vi "Prompt for Step.vi"(1 "Steps":T3[](array[typedef]), 3 "Index":i32=-1, 5 "error in (no error)":errorcluster) -> (16 "New Data Out":T3={"Type"=enum."Mouse Move", "X"=0, "Y"=0, "Delay"=0, "Key"=65, "Repeat"=0, "RClick?"=FALSE, "App/Window Name"="", "Notes"=""}, 18 "OK?":bool caption="OK", 19 "error out":errorcluster)   [LabVIEW 2023]
doc: "Prompts to enter a new step in the profile."
uses:
  CTLs/Step V3.ctl
  CTLs/Step Type V3.ctl
  <vilib>/Utility/inputDevices.llb/mouseAcquire.vi
  <vilib>/Utility/inputDevices.llb/closeMouse.vi
  <vilib>/Utility/config.llb/NI_LVConfig.lvlib
panel:
  in  "Save Default":bool
  in  "Step Notes":string
  out "Step Type Description":string
  in  "Repeat Amount":i32 min=0
  in  "Tab Control":T1(tab)
  in  "Y":i32 min=0
  in  "X":i32 min=0
  in  "Right Click?":bool
  in  "Key":u8(ring)=65
  in  "App/Window Name":string
  in  "Delay (ms)":i32=100 min=0
  in  "Step Type":T2
  in  "Cancel":bool
  in  "OK":bool caption="OK2"
  # "Left and right click at\nsame time to capture\ncurrent screen coords"
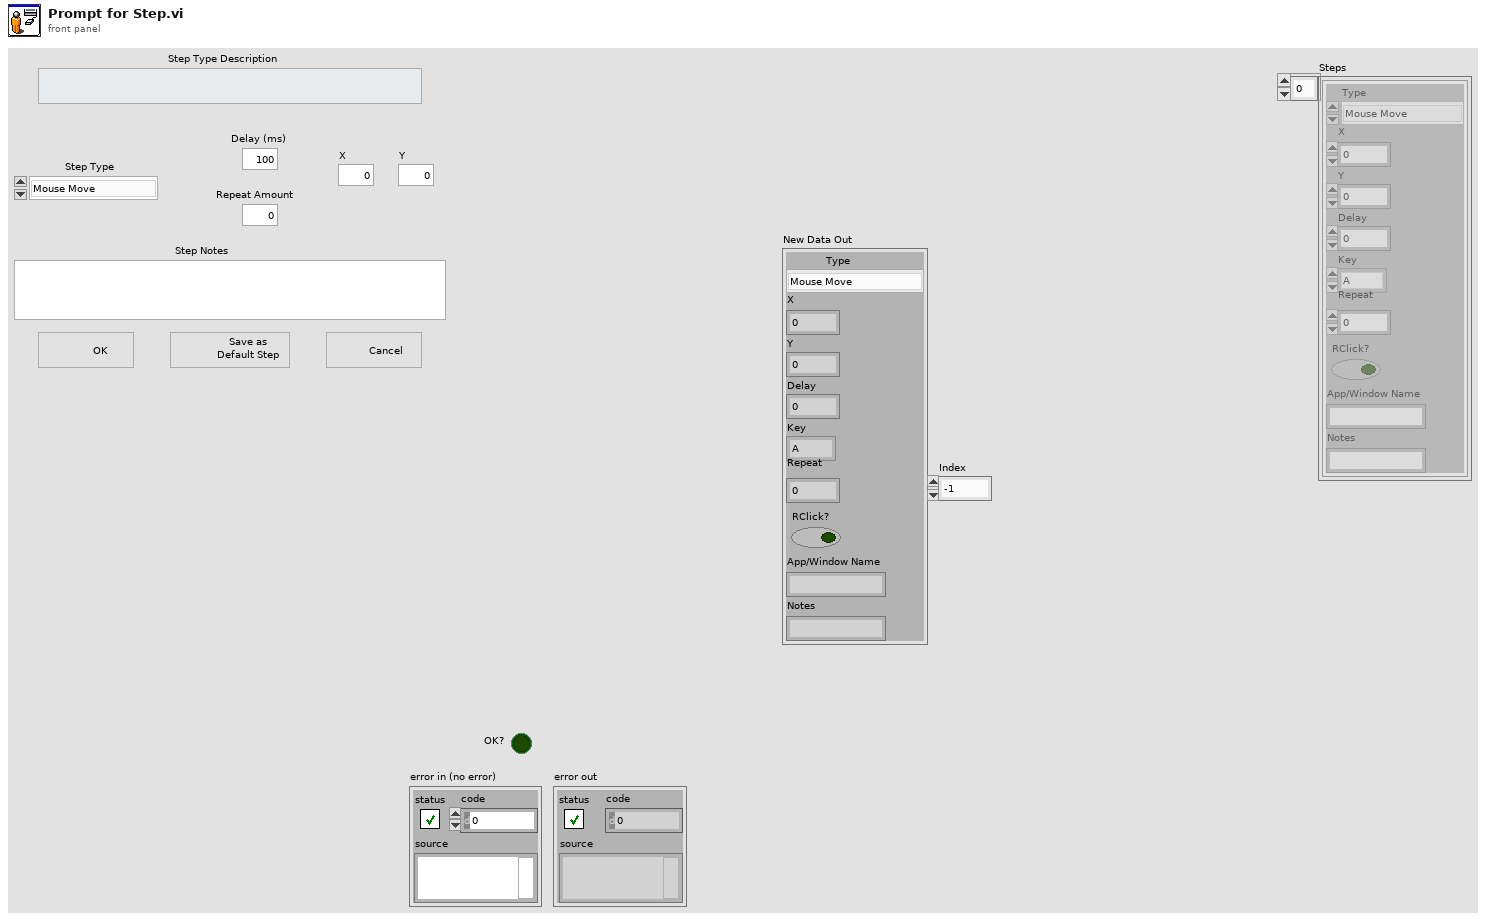
[diagram p1: front panel]
types:
  T1 = enum32{"Coords", "RClick", "Key", "A/W", "Nothing"}
  T2 = typedef "Step Type V3.ctl" = enum16{"Mouse Move", "Mouse Click", "Key Press", "Wait", "Mouse Down", "Mouse Up", "Key Down", "Key Up", "Run Application", "Maximize Window", "Restore Window", "Minimize Window", "Close Window", "Bring Window to Front", "Send Window to Back"}
  T3 = typedef "Step V3.ctl" = cluster{"Type":T2, "X":i32, "Y":i32, "Delay":i32, "Key":u8, "Repeat":i32, "RClick?":bool, "App/Window Name":string, "Notes":string}
  T4 = typedef "NI_LVConfig.lvlib/Config Data RefNum.ctl" = refnum<k1>
  T5 = cluster{"Horizontal":i32, "Vertical":i32, "Scrolling":i32}
  T6 = cluster{"button 1":bool, "button 2":bool, "button 3":bool, "button 4":bool}
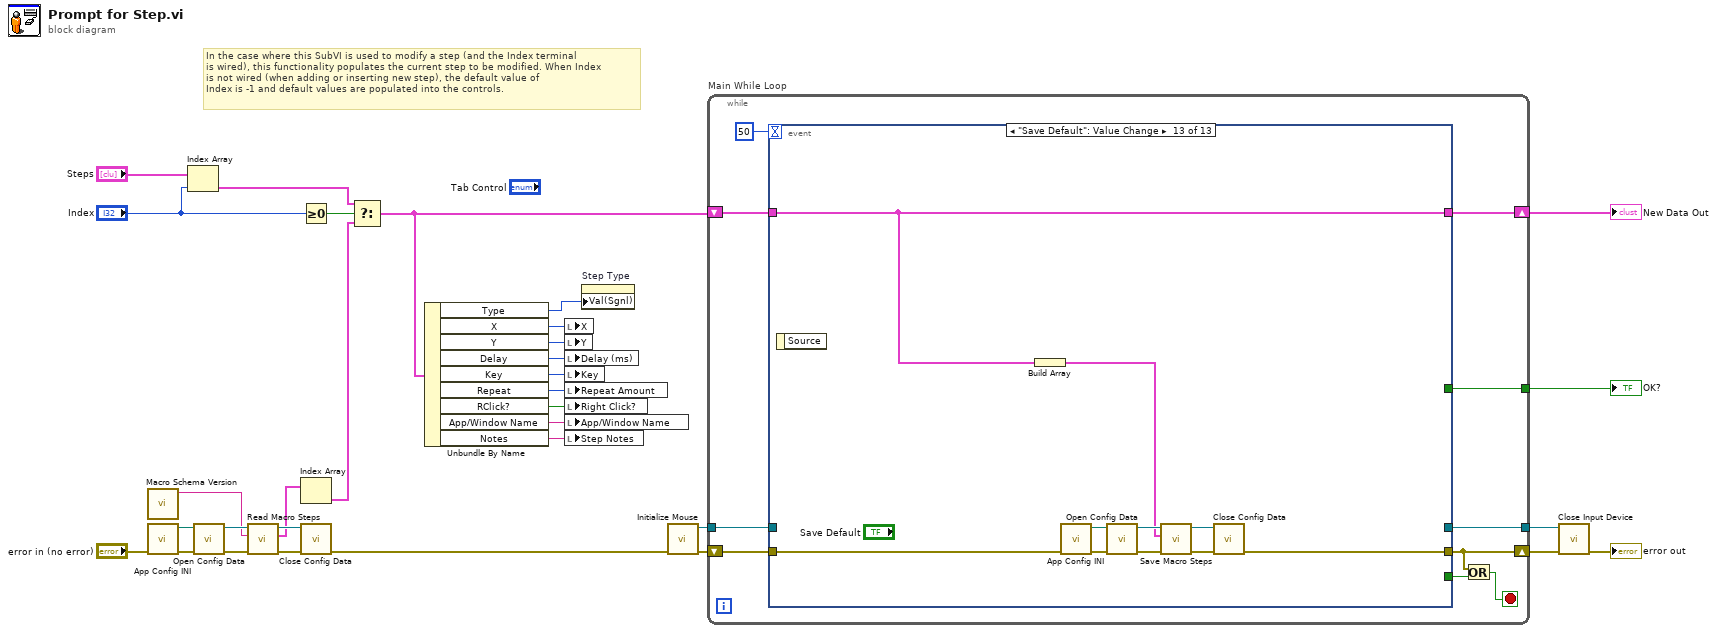
[diagram p0: block diagram]
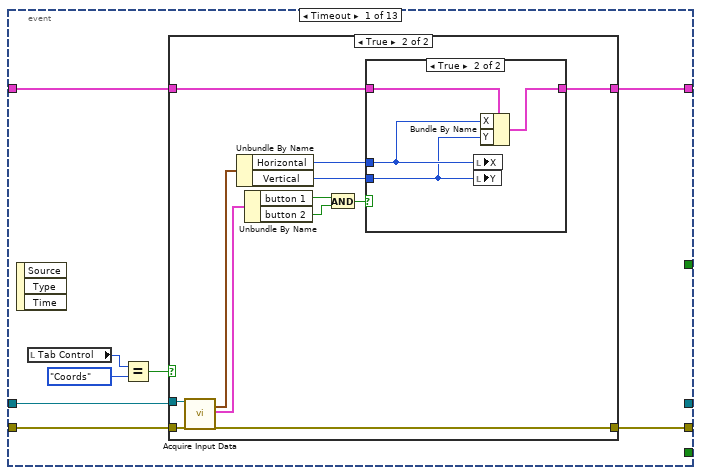
[diagram p2: hidden frame]
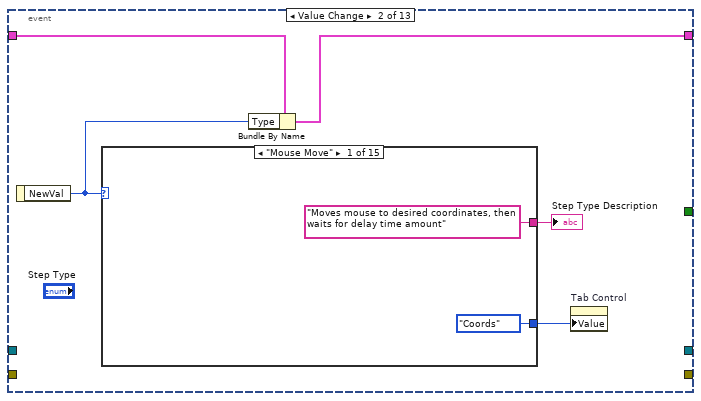
[diagram p5: hidden frame]
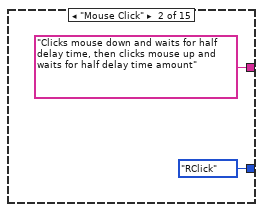
[diagram p6: hidden frame]
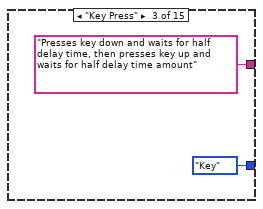
[diagram p7: hidden frame]
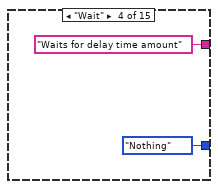
[diagram p8: hidden frame]
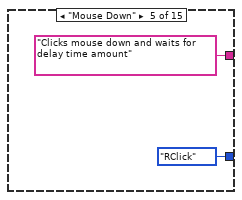
[diagram p9: hidden frame]
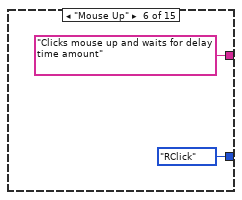
[diagram p10: hidden frame]
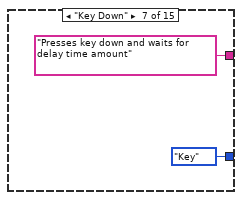
[diagram p11: hidden frame]
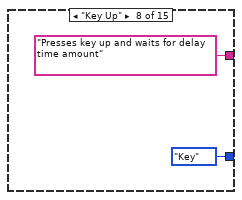
[diagram p12: hidden frame]
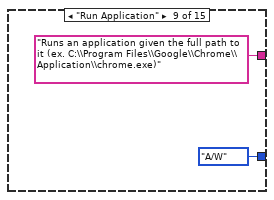
[diagram p13: hidden frame]
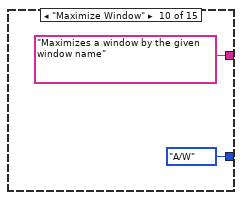
[diagram p14: hidden frame]
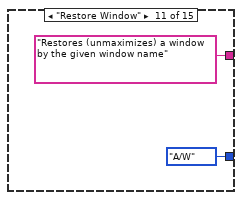
[diagram p15: hidden frame]
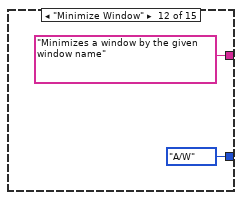
[diagram p16: hidden frame]
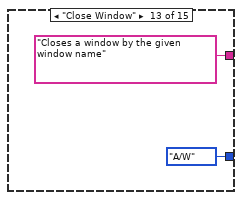
[diagram p17: hidden frame]
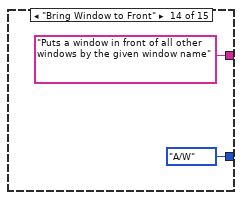
[diagram p18: hidden frame]
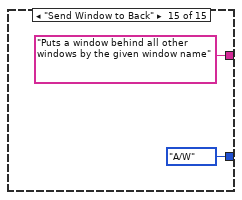
[diagram p19: hidden frame]
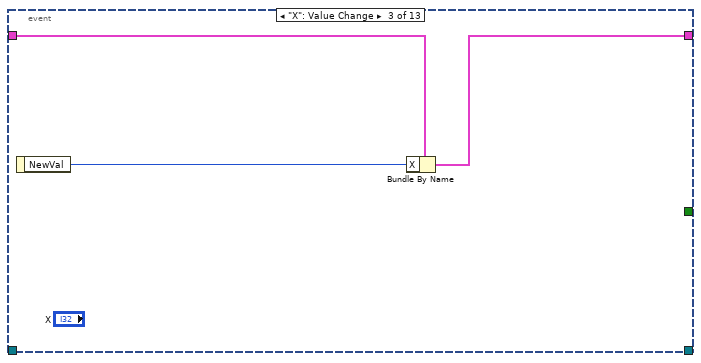
[diagram p20: hidden frame]
diagram:
  # "In the case where this SubVI is used to modify a step (and the Index terminal\nis wired), this functionality populates the current step to be modified. When Index\nis not wired (when adding or inserting new step), the default value of\nIndex is -1 and default values are populated into the controls."
  n1 = call "Macro Schema Version.vi"() -> ("Macro Schema Version"=w11:string)  [unwired: 10 in, 1 out]
  n2 = call "App Config INI.vi"("error in (no error)"="error in (no error)") -> ("error out"=w13:errorcluster, "App Config"=w14:path)  [unwired: 9 in]
  n3 = Index Array(array="Steps", index="Index") -> (element=w3:T3)
  n4 = call <vilib>:"Open Config Data.vi"("error in (no error)"=w13, "configuration file path"=w14) -> ("error out"=w10:errorcluster, "refnum"=w12:T4)  [unwired: 7 in, 1 out]
  n5 = call "Read Macro Steps.vi"("error in (no error)"=w10, "Schema Version"=w11, "refnum"=w12) -> ("error out"=w9:errorcluster, "Macro Steps"=w6:T3[], "refnum out"=w7:T4)  [unwired: 6 in]
  n6 = Greater Or Equal To 0?(x="Index") -> (x >= 0?=w4:bool)
  n7 = Index Array(array=w6) -> (element=w2:T3)  [unwired: 1 in]
  n8 = call <vilib>:"Close Config Data.vi"("error in (no error)"=w9, "refnum"=w7) -> ("error out"=w8:errorcluster)  [unwired: 8 in, 1 out]
  n9 = Select(t=w3, s=w4, f=w2) -> (s? t:f=w1:T3)
  n10 = Unbundle By Name(w1) -> ("Type"=w31:T2, "X"=w22:i32, "Y"=w16:i32, "Delay"=w21:i32, "Key"=w20:u8, "Repeat"=w19:i32, "RClick?"=w18:bool, "App/Window Name"=w17:string, "Notes"=w15:string)
  n11 = local write "X"(w22) -> ()
  n12 = local write "Y"(w16) -> ()
  n13 = local write "Delay (ms)"(w21) -> ()
  n14 = local write "Key"(w20) -> ()
  n15 = local write "Repeat Amount"(w19) -> ()
  n16 = local write "Right Click?"(w18) -> ()
  n17 = local write "App/Window Name"(w17) -> ()
  n18 = local write "Step Notes"(w15) -> ()
  n19 = property on="Step Type" class="Enum (strict)"("Val(Sgnl)"=w31) -> ()  [unwired: 2 in, 2 out]
  n20 = call <vilib>:"Initialize Mouse.vi"("error in (no error)"=w8) -> ("error out"=w29:errorcluster, "device ID"=w30:refnum<k1>)  [unwired: 9 in]
  n21 = while "Main While Loop" {
    shift-right: [w41] -> w32
    shift-left: w1 -> [w42]
    tunnel: w30 -> [w39]
    shift-right: [w35] -> w26
    shift-left: w29 -> [w38]
    tunnel: [w37] -> w27
    tunnel: [w36] -> w25
    stop <- w33 stop-if-true
    n22 = event shown="[12] \"Save Default\": Value Change" {
      selector: _ -> [_ _ _ _ _ _ _ _ _ _ _ _ _]
      dyn-events: _ -> [_ _ _ _ _ _ _ _ _ _ _ _ _]
      timeout: 50 -> [_ _ _ _ _ _ _ _ _ _ _ _ _]
      tunnel: w42 -> [w44 w74 w107 w110 w113 w116 w119 w122 w125 w128 _ w132 w138]
      tunnel: [w43 w73 w106 w109 w112 w115 w118 w121 w124 w127 _ w132 w138] -> w41
      tunnel: w39 -> [w49 _ _ _ _ _ _ _ _ _ w129 w134 _]
      tunnel: w38 -> [w50 _ _ _ _ _ _ _ _ _ w130 w135 w140]
      tunnel: [_ _ _ _ _ _ _ _ _ _ TRUE TRUE _] -> w34
      tunnel: [w46 _ _ _ _ _ _ _ _ _ w130 w135 w139] -> w35
      tunnel: [_ _ _ _ _ _ _ _ _ _ w129 w134 _] -> w37
      tunnel: [_ _ _ _ _ _ _ _ _ _ _ TRUE _] -> w36
      event Timeout {
        n23 = event-data() -> ()  [unwired: 1 in, 3 out]
        n24 = local read "Tab Control"() -> (w48:T1)
        n25 = Equal?(x=w48, y=T1."Coords" ("Tab Control")) -> (x = y?=w47:bool)
        n26 = case shown="True" w47 {
          tunnel: w50 -> [w52 w64]
          tunnel: w49 -> [_ w63]
          tunnel: [w52 w57] -> w46
          tunnel: w44 -> [w51 w54]
          tunnel: [w51 w53] -> w43
          frame False {
          }
          frame True {
            n27 = call-poly <vilib>:"Acquire Input Data.vi"("device ID"=w63, "error in (no error)"=w64) -> ("axis info"=w61:T5, "button info"=w62:T6, "error out"=w57:errorcluster)  [unwired: 14 in, 1 out]
            n28 = Unbundle By Name(w61) -> ("Horizontal"=w56:i32, "Vertical"=w55:i32)
            n29 = Unbundle By Name(w62) -> ("button 1"=w59:bool, "button 2"=w60:bool)
            n30 = And(x=w59, y=w60) -> (x .and. y?=w58:bool)
            n31 = case shown="True" w58 {
              tunnel: w56 -> [_ w67]
              tunnel: w55 -> [_ w66]
              tunnel: w54 -> [w65 w69]
              tunnel: [w65 w68] -> w53
              frame False {
              }
              frame True {
                n32 = local write "X"(w67) -> ()
                n33 = local write "Y"(w66) -> ()
                n34 = Bundle By Name(cluster=w69, "X"=w67, "Y"=w66) -> (w68:T3)
              }
            }
          }
        }
      }
      event Value Change {
        n35 = event-data() -> ("NewVal"=w72:T2)  [unwired: 1 in]
        n36 = case shown="\"Mouse Move\"" w72 {
          tunnel: ["Moves mouse to desired coordinates, then waits for delay time amount" "Clicks mouse down and waits for half delay time, then clicks mouse up and waits for half delay time amount" "Presses key down and waits for half delay time, then presses key up and waits for half delay time amount" "Waits for delay time amount" "Clicks mouse down and waits for delay time amount" "Clicks mouse up and waits for delay time amount" "Presses key down and waits for delay time amount" "Presses key up and waits for delay time amount" "Runs an application given the full path to it (ex. C:\\Program Files\\Google\\Chrome\\Application\\chrome.exe)" "Maximizes a window by the given window name" "Restores (unmaximizes) a window by the given window name" "Minimizes a window by the given window name" "Closes a window by the given window name" "Puts a window in front of all other windows by the given window name" "Puts a window behind all other windows by the given window name"] -> w71
          tunnel: [T1."Coords" ("Tab Control") T1."RClick" ("Tab Control") T1."Key" ("Tab Control") T1."Nothing" ("Tab Control") T1."RClick" ("Tab Control") T1."RClick" ("Tab Control") T1."Key" ("Tab Control") T1."Key" ("Tab Control") T1."A/W" ("Tab Control") T1."A/W" ("Tab Control") T1."A/W" ("Tab Control") T1."A/W" ("Tab Control") T1."A/W" ("Tab Control") T1."A/W" ("Tab Control") T1."A/W" ("Tab Control")] -> w70
          frame "Mouse Move" {
          }
          frame "Mouse Click" {
          }
          frame "Key Press" {
          }
          frame "Wait" {
          }
          frame "Mouse Down" {
          }
          frame "Mouse Up" {
          }
          frame "Key Down" {
          }
          frame "Key Up" {
          }
          frame "Run Application" {
          }
          frame "Maximize Window" {
          }
          frame "Restore Window" {
          }
          frame "Minimize Window" {
          }
          frame "Close Window" {
          }
          frame "Bring Window to Front" {
          }
          frame "Send Window to Back" {
          }
        }
        "Step Type Description" <- w71
        n37 = Bundle By Name(cluster=w74, "Type"=w72) -> (w73:T3)
        n38 = property on="Tab Control" class="TabCtl (strict)"("Value"=w70) -> ()  [unwired: 2 in, 2 out]
      }
      event "X": Value Change {
        n39 = event-data() -> ("NewVal"=w105:i32)  [unwired: 1 in]
        n40 = Bundle By Name(cluster=w107, "X"=w105) -> (w106:T3)
      }
      event "Y": Value Change {
        n41 = event-data() -> ("NewVal"=w108:i32)  [unwired: 1 in]
        n42 = Bundle By Name(cluster=w110, "Y"=w108) -> (w109:T3)
      }
      event "Delay (ms)": Value Change {
        n43 = event-data() -> ("NewVal"=w111:i32)  [unwired: 1 in]
        n44 = Bundle By Name(cluster=w113, "Delay"=w111) -> (w112:T3)
      }
      event "Repeat Amount": Value Change {
        n45 = event-data() -> ("NewVal"=w114:i32)  [unwired: 1 in]
        n46 = Bundle By Name(cluster=w116, "Repeat"=w114) -> (w115:T3)
      }
      event "Key": Value Change {
        n47 = event-data() -> ("NewVal"=w117:u8)  [unwired: 1 in]
        n48 = Bundle By Name(cluster=w119, "Key"=w117) -> (w118:T3)
      }
      event "Right Click?": Value Change {
        n49 = event-data() -> ("NewVal"=w120:bool)  [unwired: 1 in]
        n50 = Bundle By Name(cluster=w122, "RClick?"=w120) -> (w121:T3)
      }
      event "App/Window Name": Value Change {
        n51 = event-data() -> ("NewVal"=w123:string)  [unwired: 1 in]
        n52 = Bundle By Name(cluster=w125, "App/Window Name"=w123) -> (w124:T3)
      }
      event "Step Notes": Value Change {
        n53 = event-data() -> ("NewVal"=w126:string)  [unwired: 1 in]
        n54 = Bundle By Name(cluster=w128, "Notes"=w126) -> (w127:T3)
      }
      event "Cancel": Value Change {
        n55 = event-data() -> ()  [unwired: 1 in, 1 out]
      }
      event "OK": Value Change {
        n56 = event-data() -> ()  [unwired: 1 in, 1 out]
      }
      event "Save Default": Value Change {
        n57 = event-data() -> ()  [unwired: 1 in, 1 out]
        n58 = Build Array(w138) -> (w137:T3[])
        n59 = call "App Config INI.vi"("error in (no error)"=w140) -> ("error out"=w142:errorcluster, "App Config"=w141:path)  [unwired: 9 in]
        n60 = call <vilib>:"Open Config Data.vi"("error in (no error)"=w142, "configuration file path"=w141) -> ("error out"=w144:errorcluster, "refnum"=w143:T4)  [unwired: 7 in, 1 out]
        n61 = call "Save Macro Steps.vi"("error in (no error)"=w144, "Macro Steps"=w137, "refnum"=w143) -> ("error out"=w145:errorcluster, "refnum out"=w146:T4)  [unwired: 7 in]
        n62 = call <vilib>:"Close Config Data.vi"("error in (no error)"=w145, "refnum"=w146) -> ("error out"=w139:errorcluster)  [unwired: 8 in, 1 out]
      }
    }
    n63 = Or(x=w35, y=w34) -> (x .or. y?=w33:bool)
  }
  "OK?" <- w25
  "New Data Out" <- w32
  n64 = call-poly <vilib>:"Close Input Device.vi"("error in (no error)"=w26, "device ID"=w27) -> ("error out"=→"error out":errorcluster)  [unwired: 8 in]
